vi "test.vi"() -> ()   [LabVIEW 2019]
panel:
  in  "Stop Button 3":bool
  in  "Stop Button 2":bool
  in  "Stop Button":bool
  in  "error in (no error)":errorcluster
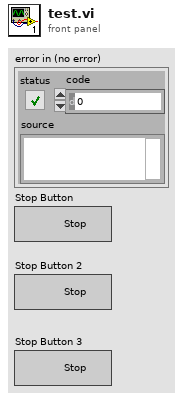
[diagram p1: front panel]
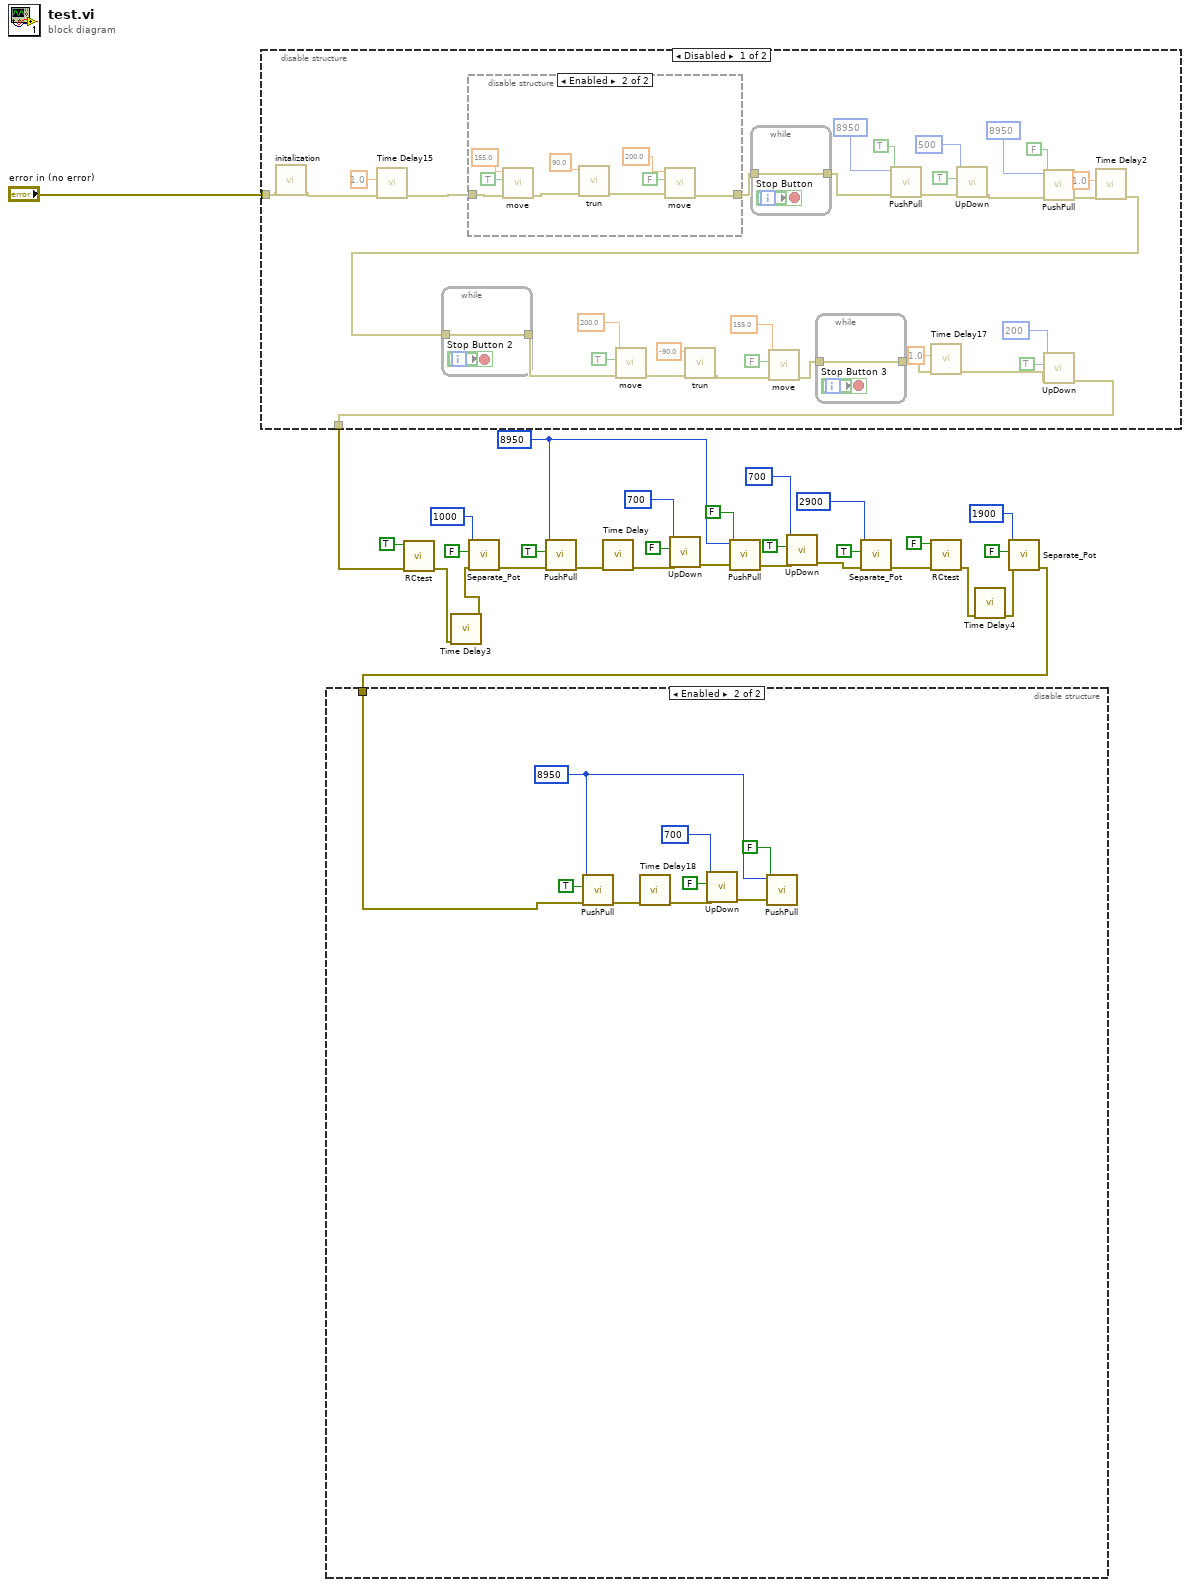
[diagram p0: block diagram]
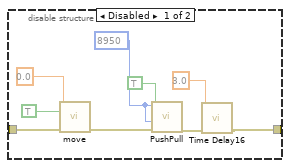
[diagram p2: hidden frame]
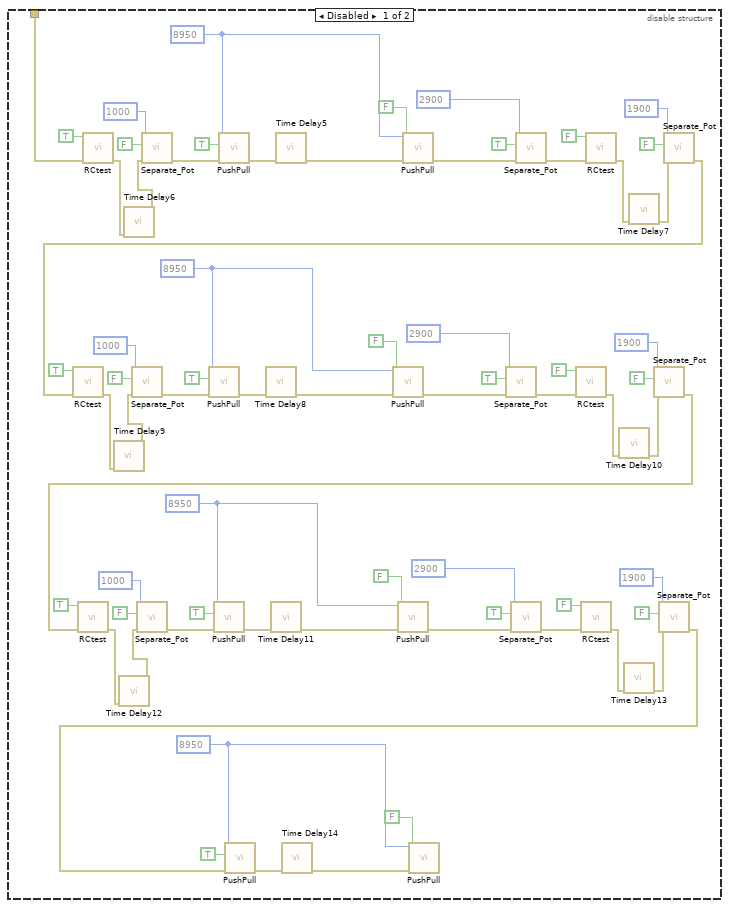
[diagram p4: hidden frame]
diagram:
  w16 = 8950 ("距離")
  n1 = disable-structure shown="Disabled" {
    disable-tunnel: "error in (no error)" -> [w49 w86]
    disable-tunnel: [w36 w86] -> w9
    frame Disabled {
      n2 = call "initalization.vi"("error in (no error)"=w49) -> ("error out"=w50:errorcluster)  [unwired: 10 in]
      n3 = call "Time Delay15"("error in (no error)"=w50, "Delay Time (s)"=1.0) -> ("error out"=w60:errorcluster)  [unwired: 9 in]
      n4 = disable-structure shown="Enabled" {
        disable-tunnel: w60 -> [w74 w85]
        disable-tunnel: [w70 w77] -> w35
        frame Disabled {
          w75 = 8950 ("距離")
          n5 = call "move.vi"("error in (no error)"=w74, "タは"=TRUE, "移動距離"=0.0) -> ("error out"=w73:errorcluster)  [unwired: 8 in]
          n6 = call "PushPull.vi"("error in (no error)"=w73, "上次位置"=w75, "轉向"=TRUE, "距離"=w75) -> ("error out"=w72:errorcluster)  [unwired: 6 in, 1 out]
          n7 = call "Time Delay16"("error in (no error)"=w72, "Delay Time (s)"=3.0) -> ("error out"=w70:errorcluster)  [unwired: 9 in]
        }
        frame Enabled {
          n8 = call "move.vi"("error in (no error)"=w85, "タは"=TRUE, "移動距離"=155.0) -> ("error out"=w81:errorcluster)  [unwired: 8 in]
          n9 = call "trun.vi"("error in (no error)"=w81, "旋轉"=90.0) -> ("error out"=w78:errorcluster)  [unwired: 9 in]
          n10 = call "move.vi"("error in (no error)"=w78, "タは"=FALSE, "移動距離"=200.0) -> ("error out"=w77:errorcluster)  [unwired: 8 in]
        }
      }
      n11 = while {
        tunnel: [w67] -> w34
        tunnel: w35 -> [w67]
        stop <- "Stop Button" stop-if-true
      }
      n12 = call "PushPull.vi"("error in (no error)"=w34, "轉向"=TRUE, "距離"=8950) -> ("error out"=w48:errorcluster)  [unwired: 7 in, 1 out]
      n13 = call "UpDown.vi"("error in (no error)"=w48, "轉向"=TRUE, "距離"=500) -> ("error out"=w43:errorcluster)  [unwired: 7 in, 1 out]
      n14 = call "PushPull.vi"("error in (no error)"=w43, "轉向"=FALSE, "距離"=8950) -> ("error out"=w42:errorcluster)  [unwired: 7 in, 1 out]
      n15 = call "Time Delay2"("error in (no error)"=w42, "Delay Time (s)"=1.0) -> ("error out"=w32:errorcluster)  [unwired: 9 in]
      n16 = while {
        tunnel: [w65] -> w33
        tunnel: w32 -> [w65]
        stop <- "Stop Button 2" stop-if-true
      }
      n17 = call "move.vi"("error in (no error)"=w33, "タは"=TRUE, "移動距離"=200.0) -> ("error out"=w58:errorcluster)  [unwired: 8 in]
      n18 = call "trun.vi"("error in (no error)"=w58, "旋轉"=-90.0) -> ("error out"=w51:errorcluster)  [unwired: 9 in]
      n19 = call "move.vi"("error in (no error)"=w51, "タは"=FALSE, "移動距離"=155.0) -> ("error out"=w31:errorcluster)  [unwired: 8 in]
      n20 = while {
        tunnel: [w63] -> w30
        tunnel: w31 -> [w63]
        stop <- "Stop Button 3" stop-if-true
      }
      n21 = call "Time Delay17"("error in (no error)"=w30, "Delay Time (s)"=1.0) -> ("error out"=w37:errorcluster)  [unwired: 9 in]
      n22 = call "UpDown.vi"("error in (no error)"=w37, "轉向"=TRUE, "距離"=200) -> ("error out"=w36:errorcluster)  [unwired: 7 in, 1 out]
    }
    frame Enabled {
    }
  }
  n23 = call "RCtest.vi"("error in (no error)"=w9, "s"=TRUE) -> ("error out"=w15:errorcluster)  [unwired: 9 in]
  n24 = call "Time Delay3"("error in (no error)"=w15) -> ("error out"=w14:errorcluster)  [unwired: 10 in]
  n25 = call "Separate_Pot.vi"("error in (no error)"=w14, "轉向"=FALSE, "距離"=1000) -> ("error out"=w26:errorcluster)  [unwired: 7 in, 1 out]
  n26 = call "PushPull.vi"("error in (no error)"=w26, "轉向"=TRUE, "距離"=w16) -> ("error out"=w24:errorcluster)  [unwired: 7 in, 1 out]
  n27 = call "Time Delay"("error in (no error)"=w24) -> ("error out"=w6:errorcluster)  [unwired: 10 in]
  n28 = call "UpDown.vi"("error in (no error)"=w6, "轉向"=FALSE, "距離"=700) -> ("error out"=w5:errorcluster)  [unwired: 7 in, 1 out]
  n29 = call "PushPull.vi"("error in (no error)"=w5, "轉向"=FALSE, "距離"=w16) -> ("error out"=w3:errorcluster)  [unwired: 7 in, 1 out]
  n30 = call "UpDown.vi"("error in (no error)"=w3, "轉向"=TRUE, "距離"=700) -> ("error out"=w2:errorcluster)  [unwired: 7 in, 1 out]
  n31 = call "Separate_Pot.vi"("error in (no error)"=w2, "轉向"=TRUE, "距離"=2900) -> ("error out"=w19:errorcluster)  [unwired: 7 in, 1 out]
  n32 = call "RCtest.vi"("error in (no error)"=w19, "s"=FALSE) -> ("error out"=w13:errorcluster)  [unwired: 9 in]
  n33 = call "Time Delay4"("error in (no error)"=w13) -> ("error out"=w12:errorcluster)  [unwired: 10 in]
  n34 = call "Separate_Pot.vi"("error in (no error)"=w12, "轉向"=FALSE, "距離"=1900) -> ("error out"=w11:errorcluster)  [unwired: 7 in, 1 out]
  n35 = disable-structure shown="Enabled" {
    disable-tunnel: w11 -> [w136 w156]
    frame Disabled {
      w88 = 8950 ("距離")
      w110 = 8950 ("距離")
      w119 = 8950 ("距離")
      w151 = 8950 ("距離")
      n36 = call "RCtest.vi"("error in (no error)"=w136, "s"=TRUE) -> ("error out"=w152:errorcluster)  [unwired: 9 in]
      n37 = call "Time Delay6"("error in (no error)"=w152) -> ("error out"=w153:errorcluster)  [unwired: 10 in]
      n38 = call "Separate_Pot.vi"("error in (no error)"=w153, "轉向"=FALSE, "距離"=1000) -> ("error out"=w139:errorcluster)  [unwired: 7 in, 1 out]
      n39 = call "PushPull.vi"("error in (no error)"=w139, "轉向"=TRUE, "距離"=w151) -> ("error out"=w141:errorcluster)  [unwired: 7 in, 1 out]
      n40 = call "Time Delay5"("error in (no error)"=w141) -> ("error out"=w142:errorcluster)  [unwired: 10 in]
      n41 = call "PushPull.vi"("error in (no error)"=w142, "轉向"=FALSE, "距離"=w151) -> ("error out"=w144:errorcluster)  [unwired: 7 in, 1 out]
      n42 = call "Separate_Pot.vi"("error in (no error)"=w144, "轉向"=TRUE, "距離"=2900) -> ("error out"=w148:errorcluster)  [unwired: 7 in, 1 out]
      n43 = call "RCtest.vi"("error in (no error)"=w148, "s"=FALSE) -> ("error out"=w154:errorcluster)  [unwired: 9 in]
      n44 = call "Time Delay7"("error in (no error)"=w154) -> ("error out"=w155:errorcluster)  [unwired: 10 in]
      n45 = call "Separate_Pot.vi"("error in (no error)"=w155, "轉向"=FALSE, "距離"=1900) -> ("error out"=w94:errorcluster)  [unwired: 7 in, 1 out]
      n46 = call "RCtest.vi"("error in (no error)"=w94, "s"=TRUE) -> ("error out"=w118:errorcluster)  [unwired: 9 in]
      n47 = call "Time Delay9"("error in (no error)"=w118) -> ("error out"=w117:errorcluster)  [unwired: 10 in]
      n48 = call "Separate_Pot.vi"("error in (no error)"=w117, "轉向"=FALSE, "距離"=1000) -> ("error out"=w131:errorcluster)  [unwired: 7 in, 1 out]
      n49 = call "PushPull.vi"("error in (no error)"=w131, "轉向"=TRUE, "距離"=w119) -> ("error out"=w129:errorcluster)  [unwired: 7 in, 1 out]
      n50 = call "Time Delay8"("error in (no error)"=w129) -> ("error out"=w128:errorcluster)  [unwired: 10 in]
      n51 = call "PushPull.vi"("error in (no error)"=w128, "轉向"=FALSE, "距離"=w119) -> ("error out"=w126:errorcluster)  [unwired: 7 in, 1 out]
      n52 = call "Separate_Pot.vi"("error in (no error)"=w126, "轉向"=TRUE, "距離"=2900) -> ("error out"=w122:errorcluster)  [unwired: 7 in, 1 out]
      n53 = call "RCtest.vi"("error in (no error)"=w122, "s"=FALSE) -> ("error out"=w116:errorcluster)  [unwired: 9 in]
      n54 = call "Time Delay10"("error in (no error)"=w116) -> ("error out"=w115:errorcluster)  [unwired: 10 in]
      n55 = call "Separate_Pot.vi"("error in (no error)"=w115, "轉向"=FALSE, "距離"=1900) -> ("error out"=w93:errorcluster)  [unwired: 7 in, 1 out]
      n56 = call "RCtest.vi"("error in (no error)"=w93, "s"=TRUE) -> ("error out"=w111:errorcluster)  [unwired: 9 in]
      n57 = call "Time Delay12"("error in (no error)"=w111) -> ("error out"=w112:errorcluster)  [unwired: 10 in]
      n58 = call "Separate_Pot.vi"("error in (no error)"=w112, "轉向"=FALSE, "距離"=1000) -> ("error out"=w98:errorcluster)  [unwired: 7 in, 1 out]
      n59 = call "PushPull.vi"("error in (no error)"=w98, "轉向"=TRUE, "距離"=w110) -> ("error out"=w100:errorcluster)  [unwired: 7 in, 1 out]
      n60 = call "Time Delay11"("error in (no error)"=w100) -> ("error out"=w101:errorcluster)  [unwired: 10 in]
      n61 = call "PushPull.vi"("error in (no error)"=w101, "轉向"=FALSE, "距離"=w110) -> ("error out"=w103:errorcluster)  [unwired: 7 in, 1 out]
      n62 = call "Separate_Pot.vi"("error in (no error)"=w103, "轉向"=TRUE, "距離"=2900) -> ("error out"=w107:errorcluster)  [unwired: 7 in, 1 out]
      n63 = call "RCtest.vi"("error in (no error)"=w107, "s"=FALSE) -> ("error out"=w113:errorcluster)  [unwired: 9 in]
      n64 = call "Time Delay13"("error in (no error)"=w113) -> ("error out"=w114:errorcluster)  [unwired: 10 in]
      n65 = call "Separate_Pot.vi"("error in (no error)"=w114, "轉向"=FALSE, "距離"=1900) -> ("error out"=w87:errorcluster)  [unwired: 7 in, 1 out]
      n66 = call "PushPull.vi"("error in (no error)"=w87, "轉向"=TRUE, "距離"=w88) -> ("error out"=w91:errorcluster)  [unwired: 7 in, 1 out]
      n67 = call "Time Delay14"("error in (no error)"=w91) -> ("error out"=w90:errorcluster)  [unwired: 10 in]
      n68 = call "PushPull.vi"("error in (no error)"=w90, "轉向"=FALSE, "距離"=w88) -> ()  [unwired: 7 in, 2 out]
    }
    frame Enabled {
      w160 = 8950 ("距離")
      n69 = call "PushPull.vi"("error in (no error)"=w156, "轉向"=TRUE, "距離"=w160) -> ("error out"=w158:errorcluster)  [unwired: 7 in, 1 out]
      n70 = call "Time Delay18"("error in (no error)"=w158) -> ("error out"=w163:errorcluster)  [unwired: 10 in]
      n71 = call "UpDown.vi"("error in (no error)"=w163, "轉向"=FALSE, "距離"=700) -> ("error out"=w164:errorcluster)  [unwired: 7 in, 1 out]
      n72 = call "PushPull.vi"("error in (no error)"=w164, "轉向"=FALSE, "距離"=w160) -> ()  [unwired: 7 in, 2 out]
    }
  }
